vi "test_simple_text.vi"(8 "error in":errorcluster) -> (0 "error out":errorcluster, 3 "text":string)   [LabVIEW 2020, in "Conformance MCP Server.lvlib"]
doc: "Conformance fixture (scenario tools-call-simple-text). Takes no arguments and returns the fixed text \"This is a simple text response for testing.\" in the output text."
uses:
  Conformance MCP Server.lvlib
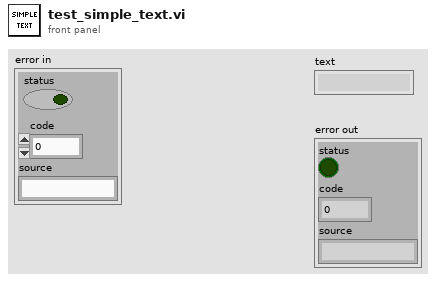
[diagram p1: front panel]
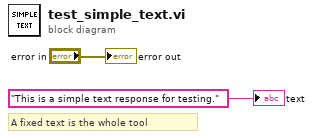
[diagram p0: block diagram]
diagram:
  # "A fixed text is the whole tool"
  "text" <- "This is a simple text response for testing." ("text")
  "error out" <- "error in"
